vi "userauth_keyboard_interactive.vi"() -> ()   [LabVIEW 2017]
doc: "Illustrates how to authenticate using keyboard-interactive authentication."
uses:
  libssh2/libssh2_session_abstract.ctl
  libssh2/libssh2_session_handshake_tcp.vi
  libssh2/libssh2_init_default.vi
  <vilib>/Utility/tcp.llb/TCP Get Raw Net Object.vi
  libssh2/libssh2_session_handshake_socket.vi
  libssh2/libssh2.lvlib
panel:
  out "authenticated":bool
  in  "username":string
  in  "hostname":string="localhost"
  out "error out":errorcluster
  # "This will be TRUE if authentication is successful."
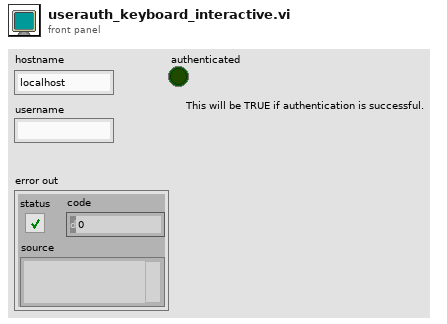
[diagram p1: front panel]
types:
  T1 = typedef "libssh2.lvlib/libssh2_session_abstract.ctl" = cluster{"send":refnum<vi>, "receive":refnum<vi>, "keyboard-interactive response":refnum<vi>}
  T2 = typedef "libssh2.lvlib/Session Refnum.ctl" = refnum<k1>
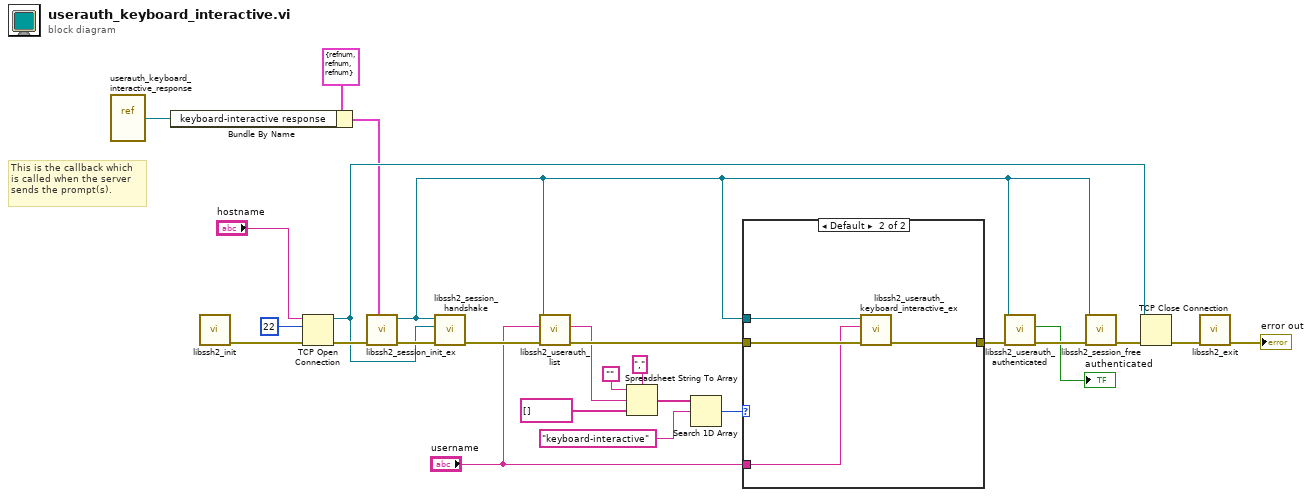
[diagram p0: block diagram]
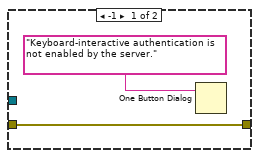
[diagram p2: hidden frame]
diagram:
  # "This is the callback which\nis called when the server\nsends the prompt(s)."
  n1 = vi-ref "userauth_keyboard_interactive_response.vi"() -> (w1:refnum<vi>)
  n2 = Bundle By Name(cluster=T1 {"send"=refnum, "receive"=refnum, "keyboard-interactive response"=refnum} ("abstract"), "keyboard-interactive response"=w1) -> (w2:T1)
  n3 = call-poly "libssh2_init.vi"() -> ("error out"=w26:errorcluster)  [unwired: 11 in]
  n4 = TCP Open Connection(address="hostname", remote port or service name=u16 22, error in (no error)=w26) -> (connection ID=w18:refnum<k5>, error out=w19:errorcluster)  [unwired: 2 in]
  n5 = call "libssh2_session_init_ex.vi"("abstract"=w2, "error in (no error)"=w19) -> ("error out"=w21:errorcluster, "session"=w5:T2)  [unwired: 8 in]
  n6 = call-poly "libssh2_session_handshake.vi"("error in (no error)"=w21, "tcp connection"=w18, "session"=w5) -> ("error out"=w17:errorcluster)  [unwired: 8 in]
  n7 = call "libssh2_userauth_list.vi"("error in (no error)"=w17, "username"="username", "session"=w5) -> ("error out"=w13:errorcluster, "supported authentication schemes"=w6:string)  [unwired: 7 in]
  n8 = Spreadsheet String To Array(delimiter (Tab)=",", format string="", spreadsheet string=w6, array type (2D Dbl)=string[] []) -> (array=w8:string[])
  n9 = Search 1D Array(1D array=w8, element="keyboard-interactive") -> (index of element=w4:i32)  [unwired: 1 in]
  n10 = case shown="Default" w4 {
    tunnel: [w28 w32] -> w16
    tunnel: w13 -> [w28 w31]
    tunnel: "username" -> [_ w30]
    tunnel: w5 -> [_ w29]
    frame -1 {
      n11 = One Button Dialog(message="Keyboard-interactive authentication is not enabled by the server.") -> ()  [unwired: 1 in, 1 out]
    }
    frame Default {
      n12 = call "libssh2_userauth_keyboard_interactive_ex.vi"("error in (no error)"=w31, "username"=w30, "session"=w29) -> ("error out"=w32:errorcluster)  [unwired: 8 in]
    }
  }
  n13 = call "libssh2_userauth_authenticated.vi"("error in (no error)"=w16, "session"=w5) -> ("error out"=w15:errorcluster, "authenticated"=→"authenticated":bool)  [unwired: 8 in]
  n14 = call "libssh2_session_free.vi"("error in (no error)"=w15, "session"=w5) -> ("error out"=w20:errorcluster)  [unwired: 9 in]
  n15 = TCP Close Connection(connection ID=w18, error in (no error)=w20) -> (error out=w23:errorcluster)  [unwired: 1 in, 1 out]
  n16 = call "libssh2_exit.vi"("error in (no error)"=w23) -> ("error out"=→"error out":errorcluster)  [unwired: 10 in]
